vi "CSV_Speichern.vi"(10 "Text":string, 11 "Datei":path) -> (0 "error out":errorcluster)   [LabVIEW 2026]
doc: "Create a NEW CSV file, write and close. Existing files are refused. Empty paths return an error without showing a dialog."
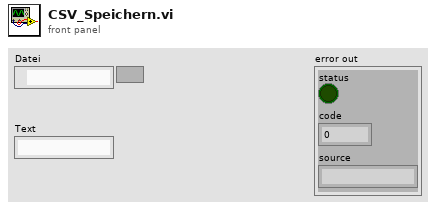
[diagram p1: front panel]
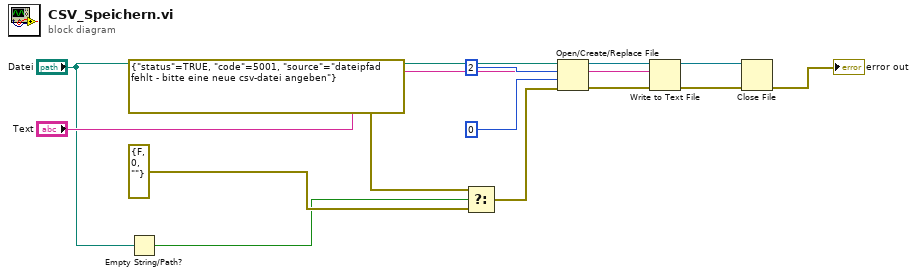
[diagram p0: block diagram]
diagram:
  n1 = Empty String/Path?(string/path="Datei") -> (empty?=w3:bool)
  n2 = Select(t=errorcluster {"status"=TRUE, "code"=5001, "source"="dateipfad fehlt - bitte eine neue csv-datei angeben"}, s=w3, f=errorcluster {"status"=FALSE, "code"=0, "source"=""}) -> (s? t:f=w6:errorcluster)
  n3 = Open/Create/Replace File(file path (use dialog)="Datei", error in=w6, operation (0:open)=2, access (0:read/write)=0) -> (refnum out=w9:refnum<file>, error out=w10:errorcluster)  [unwired: 2 in, 1 out]
  n4 = Write to Text File(file (use dialog)=w9, text="Text", error in=w10) -> (refnum out=w11:refnum<file>, error out=w12:errorcluster)  [unwired: 1 in, 1 out]
  n5 = Close File(refnum=w11, error in=w12) -> (error out=→"error out":errorcluster)  [unwired: 1 out]
